vi "Timestamp to ISO8601 UTC DateTime.vi"(9 "UTC? (F)":bool, 11 "Timestamp (now)":timestamp) -> (3 "ISO8601 String":string)   [LabVIEW 2013]
doc: "Use \"Timestamp to ISO8601 String.vi\" as a drop-in replacement.\n\nThe VI is kept for backward compatibility, but is deprecated due to confusing name."
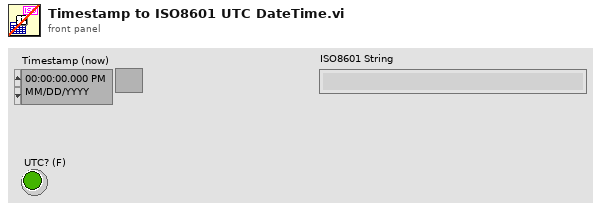
[diagram p1: front panel]
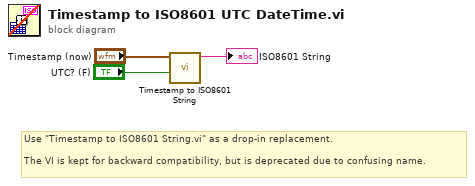
[diagram p0: block diagram]
diagram:
  # "Use \"Timestamp to ISO8601 String.vi\" as a drop-in replacement.\n\nThe VI is kept for backward compatibility, but is deprecated due to confusing name."
  n1 = call "Timestamp to ISO8601 String.vi"("UTC? (F)"="UTC? (F)", "Timestamp (now)"="Timestamp (now)") -> ("ISO8601 String"=→"ISO8601 String":string)  [unwired: 9 in]
